vi "十字路口仿真V3.2_线路优化版.vi"() -> ()   [LabVIEW 2014]
panel:
  out "t_s":dbl
  out "PW_N_R":bool
  out "PW_S_R":bool
  out "PW_E_R":bool
  out "PW_W_R":bool
  out "PW_N_G":bool
  out "PW_S_G":bool
  out "PW_E_G":bool
  out "PW_W_G":bool
  out "BK_NS_TH_R":bool
  out "BK_NS_LT_R":bool
  out "BK_EW_TH_R":bool
  out "BK_EW_LT_R":bool
  out "BK_NS_TH_G":bool
  out "BK_NS_LT_G":bool
  out "BK_EW_TH_G":bool
  out "BK_EW_LT_G":bool
  out "loop_count":dbl
  in  "停止":bool
  in  "step_ms":dbl
  out "slice_name":string
  out "cycle_no":dbl
  out "remain_s":dbl
  out "EW_LT_G":bool
  out "EW_TH_G":bool
  out "NS_LT_G":bool
  out "NS_TH_G":bool
  out "EW_LT_Y":bool
  out "EW_TH_Y":bool
  out "NS_LT_Y":bool
  out "NS_TH_Y":bool
  out "EW_LT_R":bool
  out "EW_TH_R":bool
  out "NS_LT_R":bool
  out "NS_TH_R":bool
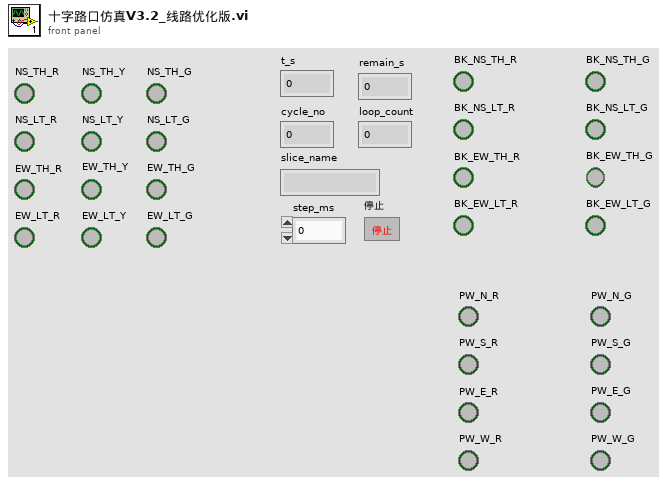
[diagram p1: front panel]
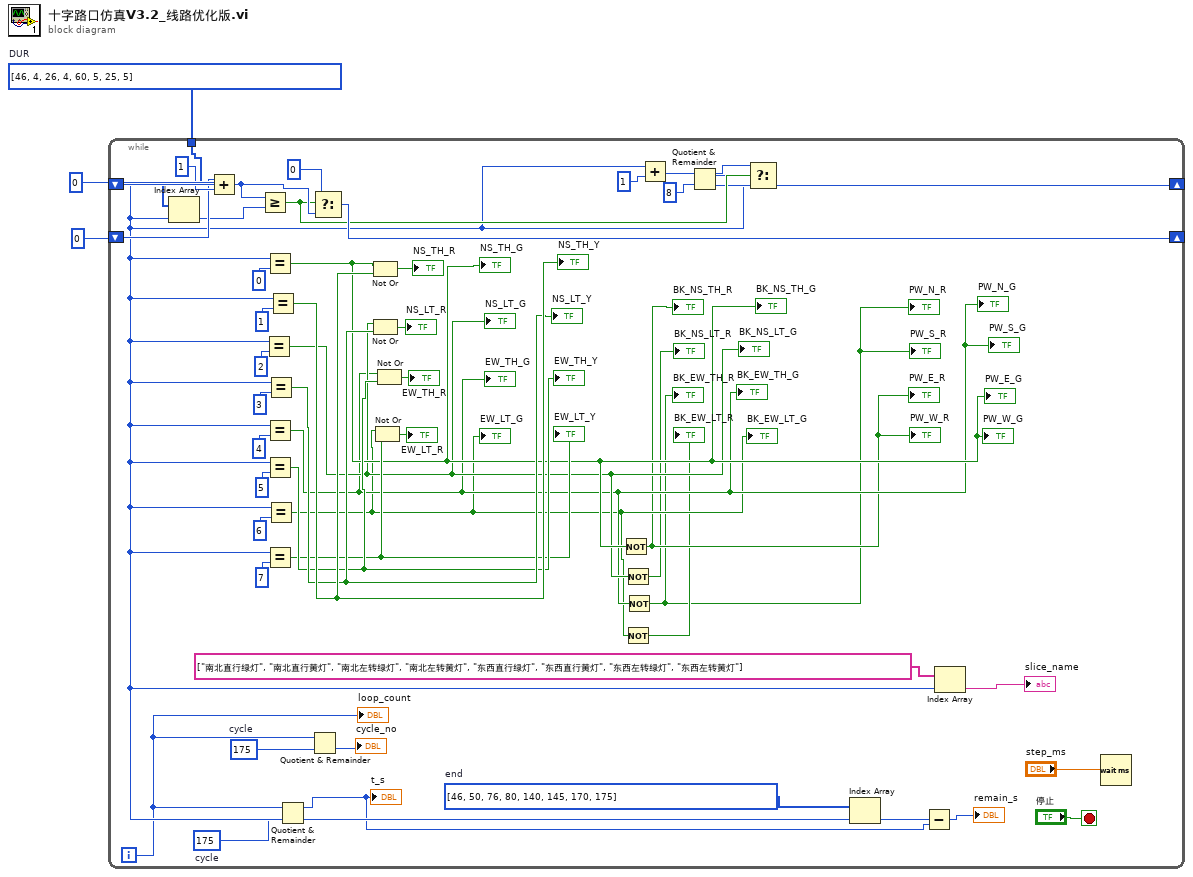
[diagram p0: block diagram]
diagram:
  w1 = i32[] [46, 4, 26, 4, 60, 5, 25, 5]  # DUR
  n1 = while {
    shift-right: [w11] -> _
    shift-left: 0 -> [w7]
    shift-right: [w17] -> _
    shift-left: 0 -> [w22]
    tunnel: w1 -> [w21]
    i -> [w5]
    stop <- "停止" stop-if-true
    w6 = 175  # cycle
    w10 = i32[] [46, 50, 76, 80, 140, 145, 170, 175]  # end
    w50 = 175  # cycle
    n2 = Index Array(array=w21, index=w7) -> (element=w20:i32)
    n3 = Add(x=w22, y=1) -> (x+y=w19:i32)
    n4 = Greater Or Equal?(x=w19, y=w20) -> (x >= y?=w13:bool)
    n5 = Equal?(x=w7, y=2) -> (x = y?=w31:bool)
    "NS_LT_G" <- w31
    "BK_NS_LT_G" <- w31
    n6 = Equal?(x=w7, y=0) -> (x = y?=w32:bool)
    "NS_TH_G" <- w32
    "BK_NS_TH_G" <- w32
    "PW_E_G" <- w32
    "PW_W_G" <- w32
    n7 = Equal?(x=w7, y=4) -> (x = y?=w30:bool)
    "EW_TH_G" <- w30
    "BK_EW_TH_G" <- w30
    "PW_N_G" <- w30
    "PW_S_G" <- w30
    n8 = Equal?(x=w7, y=5) -> (x = y?=w34:bool)
    "EW_TH_Y" <- w34
    n9 = Equal?(x=w7, y=7) -> (x = y?=w33:bool)
    "EW_LT_Y" <- w33
    n10 = Equal?(x=w7, y=3) -> (x = y?=w35:bool)
    "NS_LT_Y" <- w35
    n11 = Equal?(x=w7, y=6) -> (x = y?=w29:bool)
    "EW_LT_G" <- w29
    "BK_EW_LT_G" <- w29
    n12 = Equal?(x=w7, y=1) -> (x = y?=w36:bool)
    "NS_TH_Y" <- w36
    n13 = Quotient & Remainder(x=w5, y=w6) -> (x-y*floor(x/y)=w4:i32)  [unwired: 1 out]
    "t_s" <- w4
    n14 = Quotient & Remainder(x=w5, y=w50) -> (floor(x/y)=→"cycle_no":i32)  [unwired: 1 out]
    n15 = Select(t=0, s=w13, f=w19) -> (s? t:f=w17:i32)
    n16 = Not Or(1:w36, 2:w32) -> (0:→"NS_TH_R":bool)
    n17 = Not Or(1:w35, 2:w31) -> (0:→"NS_LT_R":bool)
    n18 = Not Or(1:w33, 2:w29) -> (0:→"EW_LT_R":bool)
    n19 = Not Or(1:w34, 2:w30) -> (0:→"EW_TH_R":bool)
    n20 = Not(x=w32) -> (.not. x?=→"BK_NS_TH_R" →"PW_E_R" →"PW_W_R":bool)
    n21 = Not(x=w31) -> (.not. x?=→"BK_NS_LT_R":bool)
    n22 = Not(x=w29) -> (.not. x?=→"BK_EW_LT_R":bool)
    n23 = Not(x=w30) -> (.not. x?=→"BK_EW_TH_R" →"PW_N_R" →"PW_S_R":bool)
    n24 = Add(x=w7, y=1) -> (x+y=w14:i32)
    n25 = Quotient & Remainder(x=w14, y=8) -> (x-y*floor(x/y)=w12:i32)  [unwired: 1 out]
    n26 = Select(t=w12, s=w13, f=w7) -> (s? t:f=w11:i32)
    n27 = Index Array(array=w10, index=w7) -> (element=w9:i32)
    n28 = Subtract(x=w9, y=w4) -> (x-y=→"remain_s":i32)
    n29 = Index Array(array=string[] ["南北直行绿灯", "南北直行黄灯", "南北左转绿灯", "南北左转黄灯", "东西直行绿灯", "东西直行黄灯", "东西左转绿灯", "东西左转黄灯"], index=w7) -> (element=→"slice_name":string)
    n30 = Wait (ms)(milliseconds to wait="step_ms") -> ()  [unwired: 1 out]
    "loop_count" <- w5
  }
